vi "Launch Server.vi"(0 "WebSocket Server Manager in":refnum<class "WebSocket Server Manager.lvclass">, 2 "Receive Server Enqueuer Handler":refnum<class "WebSocket Server-Service Enqueuer Msg.lvclass">, 5 "Listener Settings":T1={"resolve remote address (T)"=TRUE, "timeout ms (-1)"=-1, "net address"=0, "port"=6163}, 7 "Handshake timeout (5000 ms)":i32=5000, 9 "Subscriber Enqueuer":refnum<class "Message Enqueuer.lvclass">, 11 "error in (no error)":errorcluster) -> (4 "WebSocket Server Manager out":refnum<class "WebSocket Server Manager.lvclass">, 15 "error out":errorcluster)   [LabVIEW 2021, in "WebSocket Actors.lvlib" / "WebSocket Server Manager.lvclass"]
doc: "This method launches a server listening on at a specific port and interface address as detailed in the \"Listener Settings\" input. If the server is already running at that port or on the specified interface the method sends just the server enqueuer to the client. If the server is not running it will be launched."
uses:
  WebSocket Server Manager.lvclass
  C:/Program Files/National Instruments/LabVIEW 2021/vi.lib/ActorFramework/Actor/Actor.lvclass
  WebSocket Server/typedefs/Listener Settings.ctl
  <vilib>/ActorFramework/Message Enqueuer/Message Enqueuer.lvclass
  Abstract Messages/WebSocket Server-Service Enqueuer Msg/WebSocket Server-Service Enqueuer Msg.lvclass
  C:/Program Files/National Instruments/LabVIEW 2021/vi.lib/ActorFramework/Message/Message.lvclass
  WebSocket Server Manager.lvclass/WebSocket Server Manager.ctl
  WebSocket Server/WebSocket Server.lvclass
  WebSocket Server/WebSocket Server.lvclass/WebSocket Server.ctl
  Abstract Messages/WebSocket Server-Service Enqueuer Msg/WebSocket Server-Service Enqueuer Msg.lvclass/WebSocket Server-Service Enqueuer Msg.ctl
  <vilib>/ActorFramework/Message Enqueuer/Message Enqueuer.lvclass/Message Enqueuer.ctl
  WebSocket Server/Write Subscriber Enqueuer.vi
  WebSocket Server/Write Keepalive.vi
  WebSocket Server/Write Private Key.vi
  WebSocket Server/Write Certificate Chain.vi
  WebSocket Server/Write Secure.vi
  WebSocket Server/Write Load OS trusted CAs.vi
  WebSocket Server/properties/Write Handshake timeout (5000 ms).vi
  WebSocket Server/properties/Write Listener Settings.vi
  WebSocket Server/properties/Write URI.vi
  <vilib>/ActorFramework/Message Enqueuer/Enqueue.vi
  <vilib>/Utility/error.llb/Error Cluster From Error Code.vi
  <vilib>/Utility/LVClass/Get LV Class Name.vi
  <resource>/AFDebug/Generate Trace for Message.vi
  <vilib>/ActorFramework/Message Priority Queue/Priority Enqueue.vi
  <vilib>/ErrorRing/Error Ring.xnode
  <vilib>/ActorFramework/Actor/Actor.lvclass
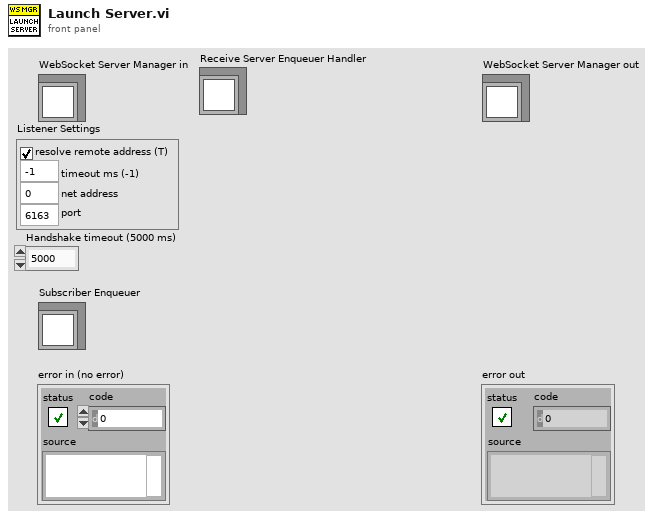
[diagram p1: front panel]
types:
  T1 = typedef "WebSocket Actors.lvlib/WebSocket Server.lvclass/Listener Settings.ctl" = cluster{"resolve remote address (T)":bool, "timeout ms (-1)":i32, "net address":u32, "port":u16}
  T2 = typedef "WebSocket Actors.lvlib/WebSocket Connection.lvclass/Keepalive.ctl" = cluster{"Enabled":bool, "Ping Interval (ms)":u32, "Ping Timeout (ms)":u32}
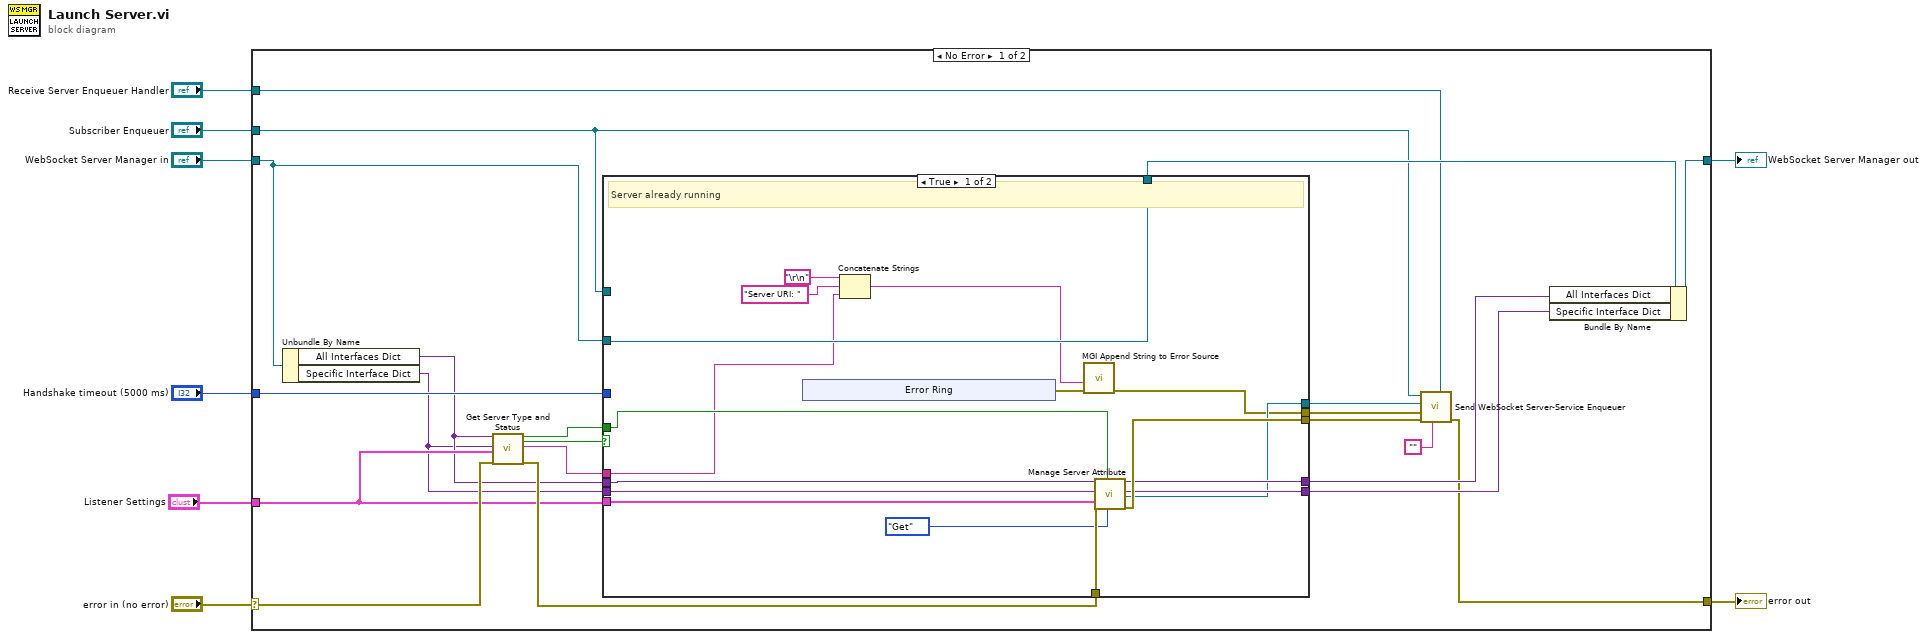
[diagram p0: block diagram]
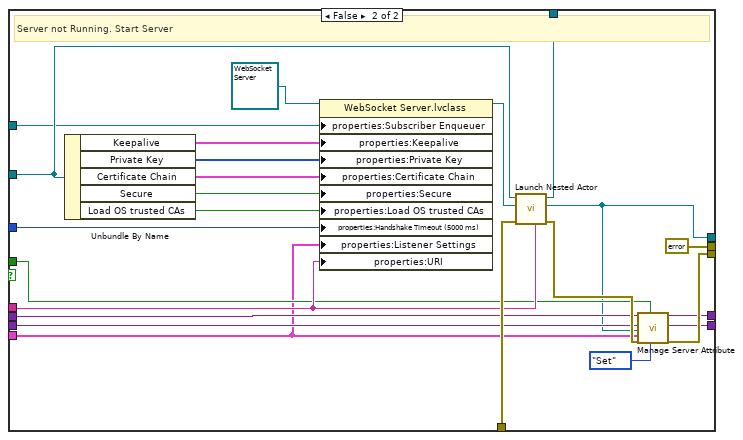
[diagram p2: hidden frame]
diagram:
  n1 = case shown="No Error" "error in (no error)" {
    selector: "error in (no error)" -> [w25 w76]
    tunnel: [w18 w76] -> w7
    tunnel: [w29 w75] -> w5
    tunnel: "WebSocket Server Manager in" -> [w28 w75]
    tunnel: "Handshake timeout (5000 ms)" -> [w26 _]
    tunnel: "Listener Settings" -> [w14 _]
    tunnel: "Subscriber Enqueuer" -> [w9 _]
    tunnel: "Receive Server Enqueuer Handler" -> [w17 _]
    frame No Error {
      n2 = Unbundle By Name(w28) -> ("All Interfaces Dict"=w13:variant, "Specific Interface Dict"=w11:variant)
      n3 = call "Get Server Type and Status.vi"("All Interfaces Dict"=w13, "Specific Interface Dict in"=w11, "Listener Settings"=w14, "error in (no error)"=w25) -> ("Is \"All Interface\" Server"=w21:bool, "Server Running"=w24:bool, "Server URI"=w16:string, "error out"=w15:errorcluster)  [unwired: 12 in]
      n4 = case shown="True" w24 {
        tunnel: w28 -> [w46 w57]
        tunnel: [w46 w72] -> w27
        tunnel: w26 -> [_ w71]
        tunnel: w14 -> [w37 w58]
        tunnel: w15 -> [w45 w70]
        tunnel: w16 -> [w31 w68]
        tunnel: [w42 w65] -> w23
        tunnel: [w38 w59] -> w12
        tunnel: [w34 errorcluster {"status"=FALSE, "code"=0, "source"=""} ("error out")] -> w22
        tunnel: w21 -> [w36 w60]
        tunnel: w13 -> [w44 w62]
        tunnel: [w41 w63] -> w20
        tunnel: [w40 w64] -> w19
        tunnel: w11 -> [w43 w61]
        tunnel: w9 -> [_ w51]
        frame True {
          # "Server already running"
          n5 = xnode "Error Ring"() -> ("error out"=w35:errorcluster)
          n6 = Concatenate Strings("\r\n", "Server URI: " ("string"), w31) -> (w30:string)
          n7 = call <userlib>:"MGI Append String to Error Source.vi"("Error In"=w35, "String to Append"=w30) -> ("Error Out"=w34:errorcluster)  [unwired: 9 in]
          n8 = call "Manage Server Attribute.vi"("All Interfaces Dict in"=w44, "Specific Interface Dict in"=w43, "Listener Settings"=w37, "error in (no error)"=w45, "Is \"All Interface\" Server"=w36, "Action"=enum16{"Set", "Get", "Delete"}."Get") -> ("All Interfaces Dict out"=w40:variant, "Specific Interface Dict out"=w41:variant, "Message Enqueuer out"=w38:refnum<class "Message Enqueuer.lvclass">, "error out"=w42:errorcluster)  [unwired: 10 in]
        }
        frame False {
          # "Server not Running. Start Server"
          n9 = Unbundle By Name(w57) -> ("Keepalive"=w56:T2, "Private Key"=w55:u8[], "Certificate Chain"=w54:cluster{"certificate":u8[]}[], "Secure"=w53:bool, "Load OS trusted CAs"=w52:bool)
          n10 = property class="WebSocket Server.lvclass"(reference=refnum<class "WebSocket Server.lvclass"> refnum ("WebSocket Actors.lvlib:WebSocket Server.lvclass"), "properties:Subscriber Enqueuer"=w51, "properties:Keepalive"=w56, "properties:Private Key"=w55, "properties:Certificate Chain"=w54, "properties:Secure"=w53, "properties:Load OS trusted CAs"=w52, "properties:Handshake Timeout (5000 ms)"=w71, "properties:Listener Settings"=w58, "properties:URI"=w68) -> (reference out=w73:refnum<class "WebSocket Server.lvclass">)  [unwired: 1 in, 1 out]
          n11 = call <vilib>:"Launch Nested Actor.vi"("Debug Alias"=w68, "error in (no error)"=w70, "Nested Actor"=w73, "Caller Actor in"=w57) -> ("error out"=w66:errorcluster, "Nested Actor's Enqueuer"=w59:refnum<class "Message Enqueuer.lvclass">, "Caller Actor out"=w72:refnum<class "WebSocket Server Manager.lvclass">)  [unwired: 5 in]
          n12 = call "Manage Server Attribute.vi"("All Interfaces Dict in"=w62, "Specific Interface Dict in"=w61, "Message Enqueuer in"=w59, "Listener Settings"=w58, "error in (no error)"=w66, "Is \"All Interface\" Server"=w60, "Action"=enum16{"Set", "Get", "Delete"}."Set") -> ("All Interfaces Dict out"=w64:variant, "Specific Interface Dict out"=w63:variant, "error out"=w65:errorcluster)  [unwired: 9 in, 1 out]
        }
      }
      n13 = call "Send WebSocket Server-Service Enqueuer.vi"("Receive Service/Server Enqueuer Handler"=w17, "Service Name"="", "error in (no error)"=w23, "Error"=w22, "WebSocket Server/Service Enqueuer"=w12, "Message Enqueuer"=w9) -> ("error out"=w18:errorcluster)  [unwired: 4 in, 1 out]
      n14 = Bundle By Name(cluster=w27, "All Interfaces Dict"=w19, "Specific Interface Dict"=w20) -> (w29:refnum<class "WebSocket Server Manager.lvclass">)
    }
    frame Error {
    }
  }
  "error out" <- w7
  "WebSocket Server Manager out" <- w5
